vi "FIFO.READ.vi"(0 "FIFO In":string, 5 "FIFO Name":string, 7 "Data Type":string, 9 "Ready for Output":bool) -> (4 "FIFO Out":string, 6 "Element":variant, 8 "Output Valid":bool)   [LabVIEW 2020]
doc: "Stand-in for an FPGA FIFO Read node with the handshake interface (FIFO In, Ready for Output -> Element, Output Valid, FIFO Out) so that a VI using it can be round-tripped through AIXML. The FIFO's configuration is given as constants on the diagram: FIFO Name (the FIFO item in the LabVIEW project) and Data Type (the element type); Element is a Variant (convert with Variant To Data in the caller). On My Computer it passes FIFO In to FIFO Out and reports Output Valid = FALSE with an empty Element. In the FPGA VI, replace each call with the real FIFO Method Node for FIFO Name and delete the constants."
panel:
  out "Data Type (cfg)":string
  out "FIFO Name (cfg)":string
  out "Ready for Output (last)":bool
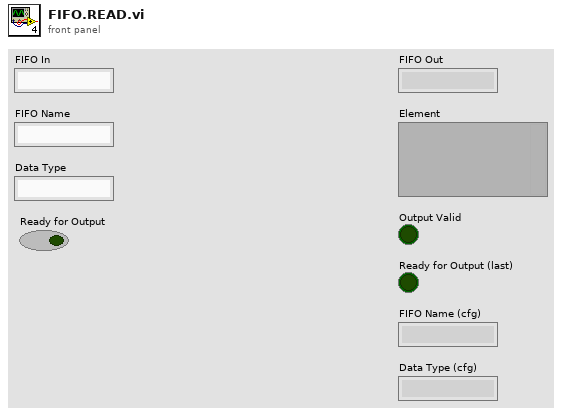
[diagram p1: front panel]
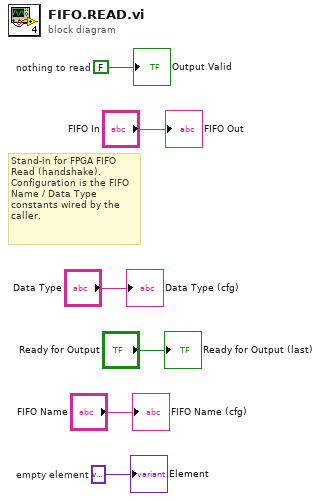
[diagram p0: block diagram]
diagram:
  w5 = variant  # empty element
  w4 = FALSE  # nothing to read
  # "Stand-in for FPGA FIFO Read (handshake). Configuration is the FIFO Name / Data Type constants wired by the caller."
  "FIFO Out" <- "FIFO In"
  "Element" <- w5
  "Output Valid" <- w4
  "Ready for Output (last)" <- "Ready for Output"
  "FIFO Name (cfg)" <- "FIFO Name"
  "Data Type (cfg)" <- "Data Type"
